vi "Process Async.vi"(6 "Client URI":refnum<class "URI.lvclass">, 9 "Secure":bool, 10 "TCP":refnum<k5>, 11 "Server in":refnum<class "Server.lvclass">) -> ()   [LabVIEW 2020, in "HTTP Server.lvlib" / "Server.lvclass"]
uses:
  Server.lvclass
  Server.lvclass/Server.ctl
  RequestTraceLog/RequestTraceLog.lvclass
  Processing/Processing.lvclass
  lv-uri/URI/URI/URI.lvclass
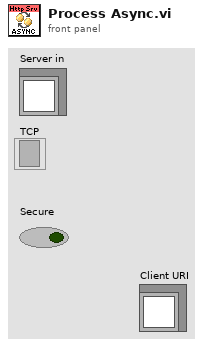
[diagram p1: front panel]
types:
  T1 = typedef "HTTP Server.lvlib/Server.lvclass/Ref Data.ctl" = cluster{"Connection Handler Map":T2, "Request Handler Map":T4, "Route Handler Map":T5, "Controller Handler Map":T6, "Controller Map":T7, "Response Handler Map":T8, "Complete Handler Map":T9, "Exception Handler Map":T10, "Connection Handler Index":u16, "Request Handler Index":u16, "Route Handler Index":u16, "Controller Handler Index":u16, "Controller Index":u16, "Response Handler Index":u16, "Complete Handler Index":u16, "Exception Handler Index":u16, "Values":refnum<class "Values.lvclass">, "Path":path, "Session Type":refnum<class "Session.lvclass">, "Session Cookie Name":string, "WebSocket Handler":refnum<class "WebSocket Handler.lvclass">, "WebSocket Handling":bool, "SSE Handler":refnum<class "SSE Handler.lvclass">, "SSE Handling":bool}
  T2 = typedef "HTTP Server.lvlib/Connection Handler Map.ctl" = map{T3, refnum<class "Connection Handler.lvclass">}
  T3 = typedef "HTTP Server.lvlib/Priority.ctl" = cluster{"Entity":u16, "Index":u16}
  T4 = typedef "HTTP Server.lvlib/Request Handler Map.ctl" = map{T3, refnum<class "Request Handler.lvclass">}
  T5 = typedef "HTTP Server.lvlib/Route Handler Map.ctl" = map{T3, refnum<class "Route Handler.lvclass">}
  T6 = typedef "HTTP Server.lvlib/Controller Handler Map.ctl" = map{T3, refnum<class "Controller Handler.lvclass">}
  T7 = typedef "HTTP Server.lvlib/Controller Map.ctl" = map{T3, refnum<class "Controller.lvclass">}
  T8 = typedef "HTTP Server.lvlib/Response Handler Map.ctl" = map{T3, refnum<class "Response Handler.lvclass">}
  T9 = typedef "HTTP Server.lvlib/Complete Handler Map.ctl" = map{T3, refnum<class "Complete Handler.lvclass">}
  T10 = typedef "HTTP Server.lvlib/Exception Handler Map.ctl" = map{T3, refnum<class "Exception Handler.lvclass">}
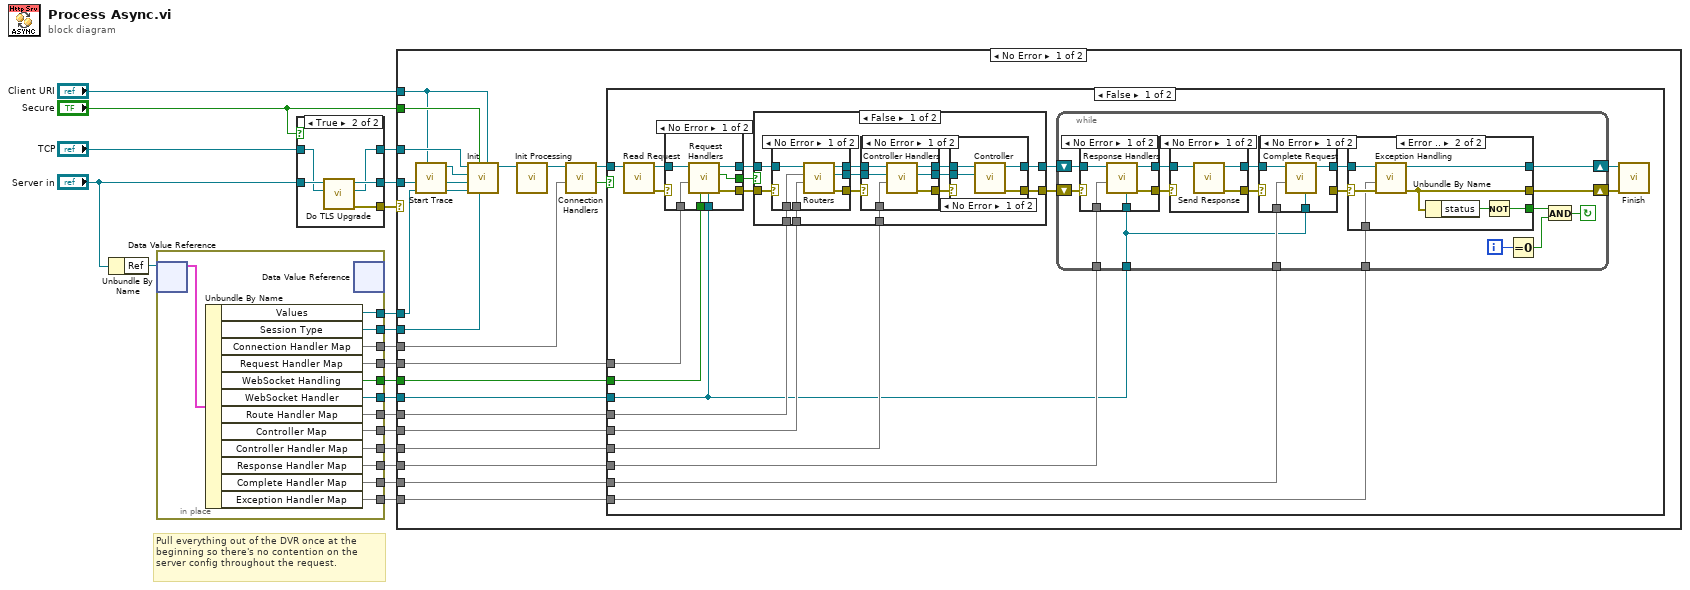
[diagram p0: block diagram]
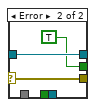
[diagram p6: hidden frame]
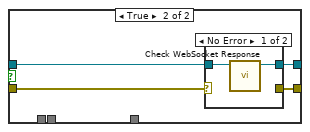
[diagram p10: hidden frame]
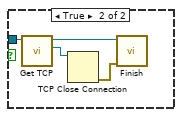
[diagram p12: hidden frame]
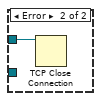
[diagram p13: hidden frame]
diagram:
  # "Pull everything out of the DVR once at the beginning so there's no contention on the server config throughout the request."
  n1 = Unbundle By Name("Server in") -> ("Ref"=w15:refnum<data-value>)
  n2 = in-place {
    in-place-border: [w32] -> w14
    in-place-border: [w31] -> w13
    in-place-border: [w24] -> w12
    in-place-border: [w30] -> w11
    in-place-border: [w29] -> w10
    in-place-border: [w28] -> w9
    in-place-border: [w27] -> w8
    in-place-border: [w26] -> w7
    in-place-border: [w25] -> w6
    in-place-border: [w23] -> w5
    in-place-border: [w22] -> w4
    in-place-border: [w21] -> w3
    n3 = in-place-dvr #1(w15) -> (w33:T1)  [unwired: 1 out]
    n4 = Unbundle By Name(w33) -> ("Values"=w21:refnum<class "Values.lvclass">, "Session Type"=w25:refnum<class "Session.lvclass">, "Connection Handler Map"=w32:T2, "Request Handler Map"=w31:T4, "WebSocket Handling"=w23:bool, "WebSocket Handler"=w22:refnum<class "WebSocket Handler.lvclass">, "Route Handler Map"=w24:T5, "Controller Map"=w30:T7, "Controller Handler Map"=w29:T6, "Response Handler Map"=w28:T8, "Complete Handler Map"=w27:T9, "Exception Handler Map"=w26:T10)
    n5 = in-place-dvr #1() -> ()  [unwired: 1 in, 2 out]
  }
  n6 = case shown="True" "Secure" {
    tunnel: "Server in" -> [w35 w40]
    tunnel: [w35 w39] -> w20
    tunnel: "TCP" -> [w34 w38]
    tunnel: [w34 w37] -> w18
    tunnel: [_ w36] -> w16
    frame False {
    }
    frame True {
      n7 = call "Do TLS Upgrade.vi"("TCP In"=w38, "Server in"=w40) -> ("error out"=w36:errorcluster, "TCP"=w37:refnum<k5>, "Server out"=w39:refnum<class "Server.lvclass">)  [unwired: 7 in]
    }
  }
  n8 = case shown="No Error" w16 {
    tunnel: w20 -> [w56 _]
    tunnel: w18 -> [w42 w183]
    tunnel: "Secure" -> [w55 _]
    tunnel: w14 -> [w54 _]
    tunnel: w13 -> [w53 _]
    tunnel: w12 -> [w52 _]
    tunnel: w11 -> [w51 _]
    tunnel: w10 -> [w50 _]
    tunnel: w9 -> [w49 _]
    tunnel: w8 -> [w48 _]
    tunnel: w7 -> [w47 _]
    tunnel: w6 -> [w46 _]
    tunnel: w5 -> [w45 _]
    tunnel: w4 -> [w44 _]
    tunnel: w3 -> [w43 _]
    tunnel: "Client URI" -> [w41 _]
    frame No Error {
      n9 = call "Start Trace.vi"("Client URI"=w41) -> ("RequestTraceLog out"=w58:refnum<class "RequestTraceLog.lvclass">)  [unwired: 9 in, 1 out]
      n10 = call "Init.vi"("Client URI"=w41, "Session"=w46, "HTTPS?"=w55, "Values"=w43, "Server"=w56, "Trace Log"=w58, "TCP"=w42) -> ("Processing out"=w57:refnum<class "Processing.lvclass">)  [unwired: 4 in]
      n11 = call "Init Processing.vi"("Processing In"=w57) -> ("Processing"=w59:refnum<class "Processing.lvclass">)  [unwired: 10 in]
      n12 = call "Connection Handlers.vi"("Connection Handler Map"=w54, "Processing In"=w59) -> ("Close?"=w60:bool, "HTTP Server.lvlib:Processing"=w61:refnum<class "Processing.lvclass">)  [unwired: 8 in]
      n13 = case shown="False" w60 {
        tunnel: w53 -> [w80 _]
        tunnel: w52 -> [w78 _]
        tunnel: w51 -> [w77 _]
        tunnel: w50 -> [w76 _]
        tunnel: w49 -> [w75 _]
        tunnel: w48 -> [w74 _]
        tunnel: w47 -> [w73 _]
        tunnel: w61 -> [w72 w182]
        tunnel: w45 -> [w66 _]
        tunnel: w44 -> [w65 _]
        frame False {
          n14 = call "Read Request.vi"("Processing In"=w72) -> ("error out"=w71:errorcluster, "HTTP Server.lvlib:Processing"=w63:refnum<class "Processing.lvclass">)  [unwired: 9 in]
          n15 = case shown="No Error" w71 {
            selector: w71 -> [_ w135]
            tunnel: w80 -> [w131 _]
            tunnel: [w130 w135] -> w79
            tunnel: w63 -> [w132 w134]
            tunnel: [w129 w134] -> w70
            tunnel: w66 -> [w128 _]
            tunnel: w65 -> [w127 _]
            tunnel: [w126 TRUE ("Early Response?")] -> w62
            frame No Error {
              n16 = call "Request Handlers.vi"("WebSocket Handler"=w127, "WebSocket Handling"=w128, "Request Handler Map"=w131, "Processing In"=w132) -> ("error out"=w130:errorcluster, "Early Response?"=w126:bool, "HTTP Server.lvlib:Processing"=w129:refnum<class "Processing.lvclass">)  [unwired: 5 in]
            }
            frame Error {
            }
          }
          n17 = case shown="False" w62 {
            tunnel: w79 -> [w148 w173]
            tunnel: w78 -> [w144 _]
            tunnel: w77 -> [w143 _]
            tunnel: w76 -> [w146 _]
            tunnel: w70 -> [w145 w174]
            tunnel: [w139 w172] -> w69
            tunnel: [w138 w171] -> w68
            frame False {
              n18 = case shown="No Error" w148 {
                selector: w148 -> [_ w156]
                tunnel: [w151 w156] -> w147
                tunnel: w145 -> [w154 w155]
                tunnel: w144 -> [w153 _]
                tunnel: w143 -> [w152 _]
                tunnel: [w150 w155] -> w142
                tunnel: [w149 _] -> w137
                frame No Error {
                  n19 = call "Routers.vi"("Controller Map"=w152, "Route Handler Map"=w153, "Processing In"=w154) -> ("error out"=w151:errorcluster, "Controller"=w149:refnum<class "Controller.lvclass">, "Processing"=w150:refnum<class "Processing.lvclass">)  [unwired: 6 in]
                }
                frame Error {
                }
              }
              n20 = case shown="No Error" w147 {
                selector: w147 -> [_ w164]
                tunnel: w146 -> [w161 _]
                tunnel: w142 -> [w162 w163]
                tunnel: [w160 w164] -> w141
                tunnel: [w159 w163] -> w140
                tunnel: w137 -> [w158 _]
                tunnel: [w157 _] -> w136
                frame No Error {
                  n21 = call "Controller Handlers.vi"("Controller Handler Map"=w161, "Controller in"=w158, "Processing In"=w162) -> ("error out"=w160:errorcluster, "Controller"=w157:refnum<class "Controller.lvclass">, "Processing"=w159:refnum<class "Processing.lvclass">)  [unwired: 6 in]
                }
                frame Error {
                }
              }
              n22 = case shown="No Error" w141 {
                selector: w141 -> [_ w170]
                tunnel: w140 -> [w168 w169]
                tunnel: [w167 w170] -> w139
                tunnel: [w166 w169] -> w138
                tunnel: w136 -> [w165 _]
                frame No Error {
                  n23 = call "Controller.vi"("Controller"=w165, "Processing In"=w168) -> ("error out"=w167:errorcluster, "Processing"=w166:refnum<class "Processing.lvclass">)  [unwired: 8 in]
                }
                frame Error {
                }
              }
            }
            frame True {
              n24 = case shown="No Error" w173 {
                selector: w173 -> [_ w178]
                tunnel: w174 -> [w176 w177]
                tunnel: [_ w178] -> w172
                tunnel: [w175 w177] -> w171
                frame No Error {
                  n25 = call "Check WebSocket Response.vi"("Processing In"=w176) -> ("Processing"=w175:refnum<class "Processing.lvclass">)  [unwired: 10 in]
                }
                frame Error {
                }
              }
            }
          }
          n26 = while {
            tunnel: w75 -> [w98]
            tunnel: w74 -> [w96]
            tunnel: w73 -> [w95]
            tunnel: w65 -> [w85]
            shift-right: [w86] -> w67
            shift-left: w69 -> [w93]
            shift-right: [w87] -> w64
            shift-left: w68 -> [w92]
            i -> [w82]
            stop <- w83 continue-if-true
            n27 = case shown="No Error" w93 {
              selector: w93 -> [_ w105]
              tunnel: w98 -> [w102 _]
              tunnel: [w101 w105] -> w97
              tunnel: w92 -> [w103 w104]
              tunnel: [w100 w104] -> w91
              tunnel: w85 -> [w99 _]
              frame No Error {
                n28 = call "Response Handlers.vi"("WebSocket Handler"=w99, "Response Handler Map"=w102, "Processing In"=w103) -> ("error out"=w101:errorcluster, "HTTP Server.lvlib:Processing"=w100:refnum<class "Processing.lvclass">)  [unwired: 7 in]
              }
              frame Error {
              }
            }
            n29 = case shown="No Error" w97 {
              selector: w97 -> [_ w110]
              tunnel: [w107 w110] -> w94
              tunnel: w91 -> [w108 w109]
              tunnel: [w106 w109] -> w90
              frame No Error {
                n30 = call "Send Response.vi"("Processing In"=w108) -> ("error out"=w107:errorcluster, "HTTP Server.lvlib:Processing"=w106:refnum<class "Processing.lvclass">)  [unwired: 9 in]
              }
              frame Error {
              }
            }
            n31 = case shown="No Error" w94 {
              selector: w94 -> [_ w116]
              tunnel: w96 -> [w114 _]
              tunnel: [_ w116] -> w89
              tunnel: w90 -> [w113 w115]
              tunnel: [w112 w115] -> w88
              tunnel: w85 -> [w111 _]
              frame No Error {
                n32 = call "Complete Request.vi"("WebSocket Handler"=w111, "Complete Handler Map"=w114, "Processing In"=w113) -> ("HTTP Server.lvlib:Processing"=w112:refnum<class "Processing.lvclass">)  [unwired: 8 in]
              }
              frame Error {
              }
            }
            n33 = case shown="Error .." w89 {
              selector: w89 -> [w118 w124]
              tunnel: w95 -> [_ w123]
              tunnel: w88 -> [w117 w125]
              tunnel: [w117 w122] -> w87
              tunnel: [w118 w121] -> w86
              tunnel: [_ w119] -> w84
              frame No Error {
              }
              frame Error {
                n34 = call "Exception Handling.vi"("error in (no error)"=w124, "Exception Handler Map"=w123, "Processing In"=w125) -> ("error out"=w121:errorcluster, "HTTP Server.lvlib:Processing"=w122:refnum<class "Processing.lvclass">)  [unwired: 7 in]
                n35 = Unbundle By Name(w121) -> ("status"=w120:bool)
                n36 = Not(x=w120) -> (.not. x?=w119:bool)
              }
            }
            n37 = Equal To 0?(x=w82) -> (x = 0?=w81:bool)
            n38 = And(x=w84, y=w81) -> (x .and. y?=w83:bool)
          }
          n39 = call "Finish.vi"("error in (no error)"=w67, "Processing"=w64) -> ()  [unwired: 10 in]
        }
        frame True {
          n40 = call "Get TCP.vi"("Processing in"=w182) -> ("TCP"=w180:refnum<k5>, "Processing out"=w181:refnum<class "Processing.lvclass">)  [unwired: 9 in]
          n41 = TCP Close Connection(connection ID=w180) -> (error out=w179:errorcluster)  [unwired: 2 in, 1 out]
          n42 = call "Finish.vi"("error in (no error)"=w179, "Processing"=w181) -> ()  [unwired: 10 in]
        }
      }
    }
    frame Error {
      n43 = TCP Close Connection(connection ID=w183) -> ()  [unwired: 2 in, 2 out]
    }
  }
